vi "Construct URI.vi"(6 "Arguments":cluster{"key":string, "value":string}[](array[cluster]), 8 "path":string, 9 "port":string, 10 "address":string, 11 "protocol":string) -> (3 "URI":string="opc.tcp://localhost:49580")   [LabVIEW 2013, in "URI.lvlib"]
uses:
  URI.lvlib
  <vilib>/regexp/Match Regular Expression.xnode
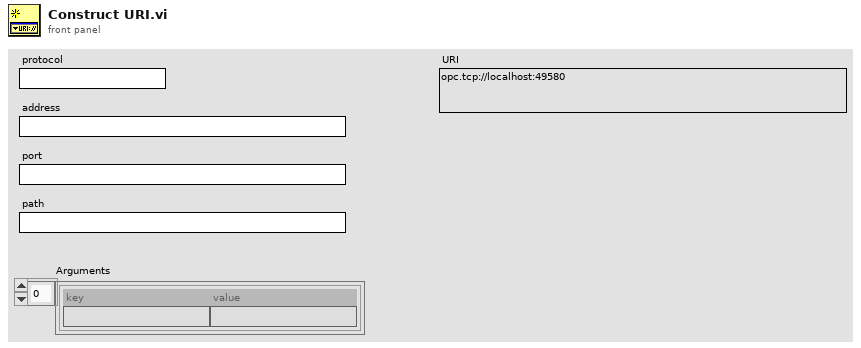
[diagram p1: front panel]
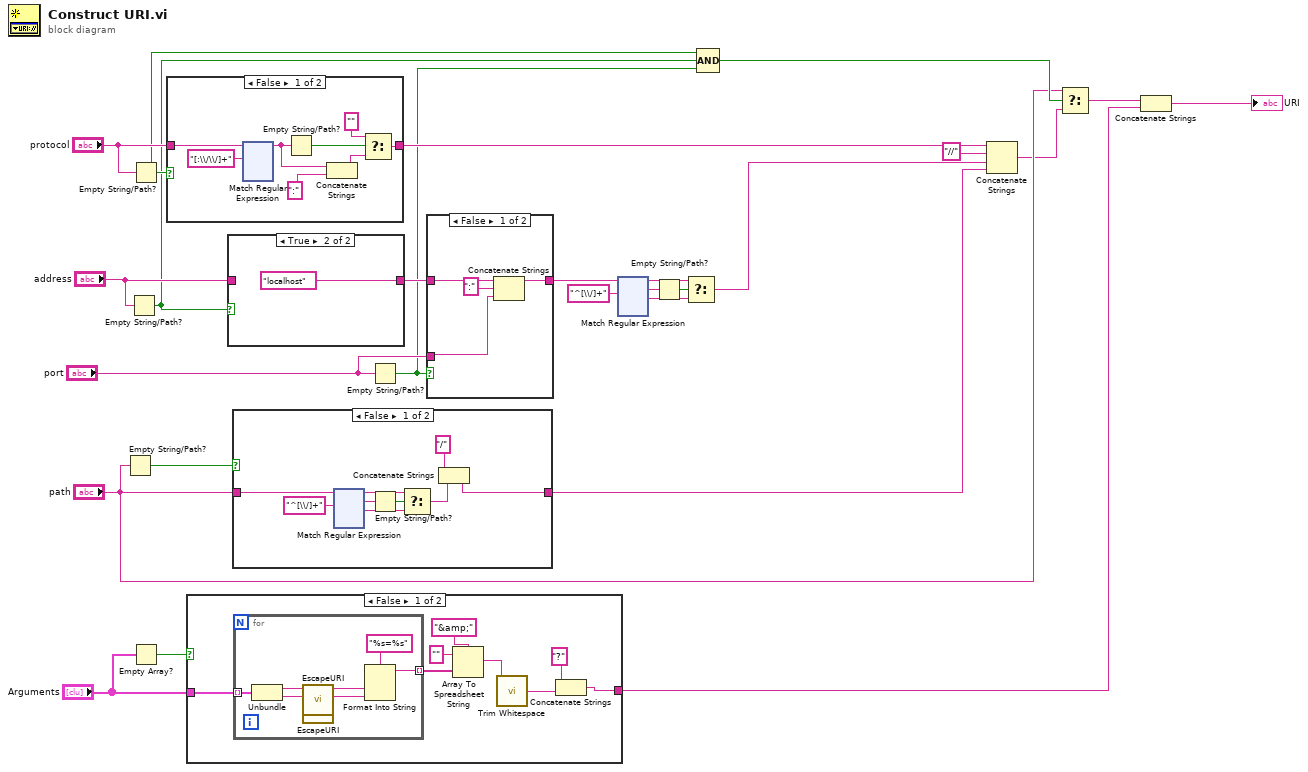
[diagram p0: block diagram]
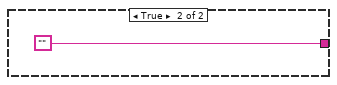
[diagram p2: hidden frame]
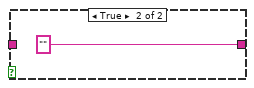
[diagram p6: hidden frame]
diagram:
  n1 = Empty String/Path?(string/path="path") -> (empty?=w3:bool)
  n2 = Empty String/Path?(string/path="address") -> (empty?=w4:bool)
  n3 = Empty String/Path?(string/path="protocol") -> (empty?=w21:bool)
  n4 = Empty Array?(array="Arguments") -> (empty?=w8:bool)
  n5 = case shown="False" w21 {
    tunnel: "protocol" -> [w33 _]
    tunnel: [w30 "" ("t")] -> w25
    frame False {
      n6 = xnode "Match Regular Expression"("input string"=w33, "regular expression"="[:\\/\\/]+") -> ("before match"=w28:string)  [unwired: 4 in, 4 out]
      n7 = Empty String/Path?(string/path=w28) -> (empty?=w32:bool)
      n8 = Concatenate Strings(w28, ":" ("t")) -> (w29:string)
      n9 = Select(t="", s=w32, f=w29) -> (s? t:f=w30:string)
    }
    frame True {
    }
  }
  n10 = case shown="False" w8 {
    tunnel: "Arguments" -> [w157 _]
    tunnel: [w150 ""] -> w7
    frame False {
      n11 = for {
        tunnel: w157 -> [w164] mode=indexing
        tunnel: [w162] -> w156 mode=indexing
        n12 = Unbundle(w164) -> ("key"=w161:string, "value"=w160:string)
        n13 = call "EscapeURI.vi"("URI"=w161) -> ("Escaped URI"=w158:string)  [unwired: 10 in]
        n14 = call "EscapeURI.vi"("URI"=w160) -> ("Escaped URI"=w159:string)  [unwired: 10 in]
        n15 = Format Into String(format string="%s=%s", w158, w159) -> (resulting string=w162:string)  [unwired: 2 in, 1 out]
      }
      n16 = Array To Spreadsheet String(delimiter (Tab)="&amp;", array=w156, 3:"" ("format string")) -> (spreadsheet string=w153:string)
      n17 = call <vilib>:"Trim Whitespace.vi"("string"=w153) -> ("trimmed string"=w151:string)  [unwired: 1 in]
      n18 = Concatenate Strings("?" ("t"), w151) -> (w150:string)
    }
    frame True {
    }
  }
  n19 = case shown="True" w4 {
    tunnel: [w166 "localhost" ("t")] -> w23
    tunnel: "address" -> [w166 _]
    frame False {
    }
    frame True {
    }
  }
  n20 = case shown="False" w3 {
    tunnel: "path" -> [w169 w291]
    tunnel: [w175 w291] -> w22
    frame False {
      n21 = xnode "Match Regular Expression"("input string"=w169, "regular expression"="^[\\/]+") -> ("before match"=w172:string, "whole match"=w171:string, "after match"=w174:string)  [unwired: 4 in, 2 out]
      n22 = Empty String/Path?(string/path=w171) -> (empty?=w173:bool)
      n23 = Select(t=w172, s=w173, f=w174) -> (s? t:f=w168:string)
      n24 = Concatenate Strings("/" ("t"), w168) -> (w175:string)
    }
    frame True {
    }
  }
  n25 = Empty String/Path?(string/path="port") -> (empty?=w20:bool)
  n26 = case shown="False" w20 {
    tunnel: "port" -> [w292 _]
    tunnel: w23 -> [w295 w296]
    tunnel: [w294 w296] -> w12
    frame False {
      n27 = Concatenate Strings(w295, ":" ("t"), w292) -> (w294:string)
    }
    frame True {
    }
  }
  n28 = xnode "Match Regular Expression"("input string"=w12, "regular expression"="^[\\/]+") -> ("before match"=w14:string, "whole match"=w15:string, "after match"=w11:string)  [unwired: 4 in, 2 out]
  n29 = Empty String/Path?(string/path=w15) -> (empty?=w13:bool)
  n30 = Select(t=w14, s=w13, f=w11) -> (s? t:f=w1:string)
  n31 = Compound Arithmetic op=AND(w21, w4, w20) -> (w19:bool)
  n32 = Concatenate Strings(w25, "//" ("t"), w1, w22) -> (w17:string)
  n33 = Select(t="path", s=w19, f=w17) -> (s? t:f=w6:string)
  n34 = Concatenate Strings(w6, w7) -> (→"URI":string)
